vi "Find All Actors In Project.vi"(8 "error in (no error)":errorcluster, 9 "Include Dependencies?":bool, 11 "Message Maker in":refnum<class "Message Maker.lvclass">) -> (0 "error out":errorcluster, 2 "Actor Classes":refnum<vi>[](array[refnum]), 3 "Message Maker out":refnum<class "Message Maker.lvclass">)   [LabVIEW 2023, in "Message Maker.lvclass"]
doc: "Finds all actors in the project\n\nAuthor: Derek Trepanier\nCopyright: MGI 2015"
uses:
  Message Maker.lvclass
  Messages Map.ctl
  Message Details.ctl
  Message Type.ctl
  Message Maker.lvclass/Message Maker.ctl
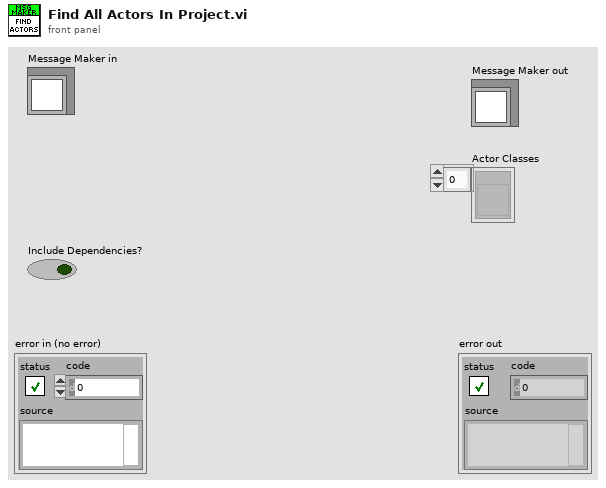
[diagram p1: front panel]
types:
  T1 = typedef "Message Maker.lvclass/Messages Map.ctl" = map{string, T2}
  T2 = typedef "Message Maker.lvclass/Message Details.ctl" = cluster{"Message Ref":refnum<vi>, "Message Type":T3}
  T3 = typedef "Message Maker.lvclass/Message Type.ctl" = enum16{"Standard", "Async"}
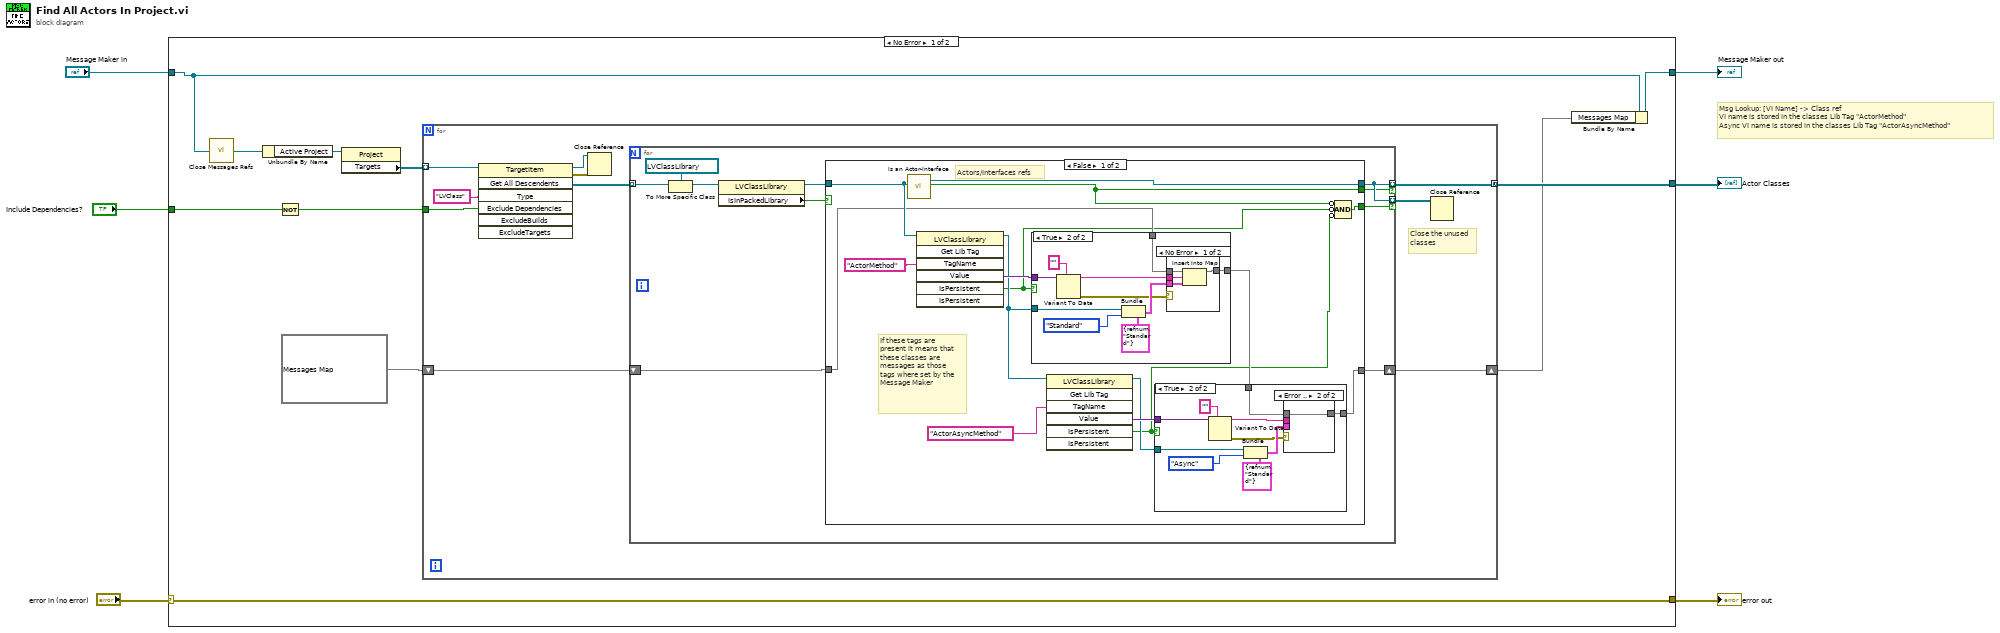
[diagram p0: block diagram]
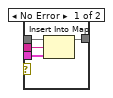
[diagram p5: hidden frame]
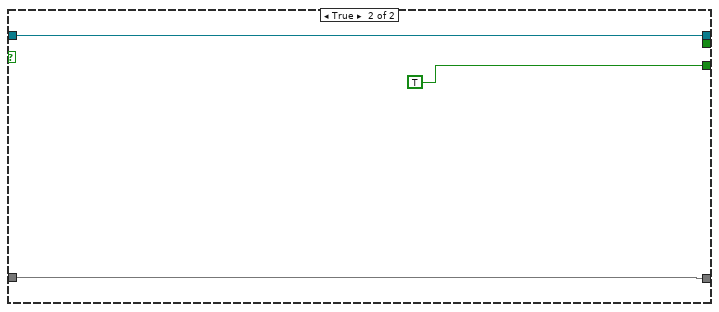
[diagram p6: hidden frame]
diagram:
  # "Msg Lookup: [VI Name] -> Class ref\nVI name is stored in the classes Lib Tag \"ActorMethod\"\nAsync VI name is stored in the classes Lib Tag \"ActorAsyncMethod\""
  n1 = case shown="No Error" "error in (no error)" {
    selector: "error in (no error)" -> [w17 w89]
    tunnel: [w17 w89] -> w5
    tunnel: "Include Dependencies?" -> [w15 _]
    tunnel: [w14 _] -> w3
    tunnel: "Message Maker in" -> [w8 w88]
    tunnel: [w12 w88] -> w1
    frame No Error {
      n2 = call "Close Messages Refs.vi"("Message Maker in"=w8) -> ("Message Maker out"=w7:refnum<class "Message Maker.lvclass">)
      n3 = Unbundle By Name(w7) -> ("Active Project"=w13:refnum<vi>)
      n4 = Not(x=w15) -> (.not. x?=w11:bool)
      n5 = property class="Project"(reference=w13) -> ("Targets"=w16:refnum<vi>[])  [unwired: 1 in, 2 out]
      n6 = for {
        tunnel: w16 -> [w27] mode=indexing
        tunnel: w11 -> [w25]
        tunnel: [w23] -> w14 mode=concatenating
        shift-right: [w18] -> w9
        shift-left: T1 {} ("Message Map") -> [w19]
        # "Close the unused classes"
        n7 = invoke class="TargetItem" method="Get All Descendents"(reference=w27, "Type"="LVClass", "Exclude Dependencies"=w25) -> (reference out=w20:refnum<vi>, error out=w21:errorcluster, "All Descendents"=w24:refnum<vi>[])  [unwired: 4 in, 4 out]
        n8 = Close Reference(reference=w20, error in (no error)=w21) -> ()  [unwired: 1 out]
        n9 = for {
          tunnel: w24 -> [w37] mode=indexing
          tunnel: [w33] -> w23 mode=indexing if=w32
          tunnel: [w33] -> w22 mode=indexing if=w35
          shift-right: [w28] -> w18
          shift-left: w19 -> [w29]
          n10 = To More Specific Class(target class=refnum<vi> refnum ("reference out"), reference=w37) -> (specific class reference=w34:refnum<vi>)  [unwired: 1 in, 1 out]
          n11 = property class="LVClassLibrary"(reference=w34) -> (reference out=w31:refnum<vi>, "IsInPackedLibrary"=w30:bool)  [unwired: 1 in, 1 out]
          n12 = case shown="False" w30 {
            tunnel: [w50 TRUE] -> w35
            tunnel: [w49 w87] -> w33
            tunnel: [w48 _] -> w32
            tunnel: w31 -> [w47 w87]
            tunnel: w29 -> [w44 w85]
            tunnel: [w40 w85] -> w28
            frame False {
              # "If these tags are present it means that these classes are messages as those tags where set by the Message Maker"
              # "Actors/Interfaces refs"
              n13 = call "Is an Actor-Interface.vi"("Class in"=w47) -> ("Class out"=w49:refnum<vi>, "Is Actor/Interface?"=w48:bool)  [unwired: 14 in, 3 out]
              n14 = invoke class="LVClassLibrary" method="Get Lib Tag"(reference=w47, "TagName"="ActorMethod" ("Tag Name")) -> (reference out=w43:refnum<vi>, "Value"=w51:variant, "IsPersistent"=w38:bool)  [unwired: 5 in, 4 out]
              n15 = case shown="True" w38 {
                tunnel: w51 -> [_ w63]
                tunnel: w44 -> [w53 w61]
                tunnel: w43 -> [_ w58]
                tunnel: [w53 w55] -> w42
                frame False {
                }
                frame True {
                  n16 = Variant To Data(type="" ("Tag Name"), Variant=w63) -> (data=w60:string, error out=w54:errorcluster)  [unwired: 1 in]
                  n17 = Bundle(cluster=T2 {"Message Ref"=refnum, "Message Type"=enum."Standard"} ("Message Details"), "Message Ref"=w58, "Message Type"=Message_Type."Standard") -> (w56:T2)
                  n18 = case shown="No Error" w54 {
                    tunnel: w61 -> [w67 w68]
                    tunnel: w60 -> [w66 _]
                    tunnel: w56 -> [w65 _]
                    tunnel: [w64 w68] -> w55
                    frame No Error {
                      n19 = Insert Into Map(map in=w67, key=w66, value=w65) -> (map out=w64:T1)  [unwired: 2 out]
                    }
                    frame Error {
                    }
                  }
                }
              }
              n20 = invoke class="LVClassLibrary" method="Get Lib Tag"(reference=w43, "TagName"="ActorAsyncMethod" ("Tag Name")) -> (reference out=w41:refnum<vi>, "Value"=w45:variant, "IsPersistent"=w39:bool)  [unwired: 5 in, 4 out]
              n21 = case shown="True" w39 {
                tunnel: w45 -> [_ w79]
                tunnel: w42 -> [w69 w77]
                tunnel: w41 -> [_ w74]
                tunnel: [w69 w71] -> w40
                frame False {
                }
                frame True {
                  n22 = Variant To Data(type="" ("Tag Name"), Variant=w79) -> (data=w76:string, error out=w70:errorcluster)  [unwired: 1 in]
                  n23 = Bundle(cluster=T2 {"Message Ref"=refnum, "Message Type"=enum."Standard"} ("Message Details"), "Message Ref"=w74, "Message Type"=Message_Type."Async") -> (w72:T2)
                  n24 = case shown="Error .." w70 {
                    tunnel: w77 -> [w83 w84]
                    tunnel: w76 -> [w82 _]
                    tunnel: w72 -> [w81 _]
                    tunnel: [w80 w84] -> w71
                    frame No Error {
                      n25 = Insert Into Map(map in=w83, key=w82, value=w81) -> (map out=w80:T1)  [unwired: 2 out]
                    }
                    frame Error {
                    }
                  }
                }
              }
              n26 = Compound Arithmetic op=AND(invert w48, invert w38, invert w39) -> (w50:bool)
            }
            frame True {
            }
          }
        }
        n27 = Close Reference(reference=w22) -> ()  [unwired: 1 in, 1 out]
      }
      n28 = Bundle By Name(cluster=w8, "Messages Map"=w9) -> (w12:refnum<class "Message Maker.lvclass">)
    }
    frame Error {
    }
  }
  "error out" <- w5
  "Actor Classes" <- w3
  "Message Maker out" <- w1
